vi "Abort On Stop.vi"(8 "error in":errorcluster, 11 "Sequence Executor in":refnum<class "Sequence Executor.lvclass">) -> (0 "error out":errorcluster, 3 "Sequence Executor out":refnum<class "Sequence Executor.lvclass">)   [LabVIEW 2026, in "Sequence Executor.lvclass"]
doc: "Stop Core hook (series, before Call Parent). If a sequence is running when the actor is told to stop, aborts it first so safe setpoints reach the rig before the nested rig actor stops. No-op when nothing is running."
uses:
  Sequence Executor.lvclass
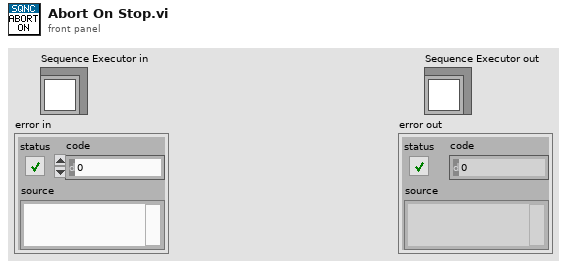
[diagram p1: front panel]
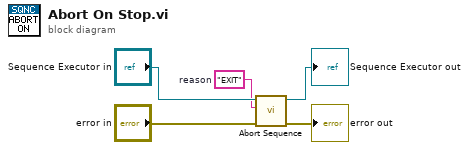
[diagram p0: block diagram]
diagram:
  w4 = "EXIT"  # reason
  n1 = call "Abort Sequence.vi"("error in"="error in", "reason"=w4, "Sequence Executor in"="Sequence Executor in") -> ("error out"=→"error out":errorcluster, "Sequence Executor out"=→"Sequence Executor out":refnum<class "Sequence Executor.lvclass">)  [unwired: 7 in]
